vi "GOOP400_ConfigurationMemory.vi"(1 "OptionsIn":T1, 5 "error in (no error)":errorcluster, 6 "Action":enum16{"Read", "Load", "Save"}(ring)) -> (15 "OptionsOut":T1, 19 "error out":errorcluster)   [LabVIEW 2020]
uses:
  GOOP400_Options.ctl
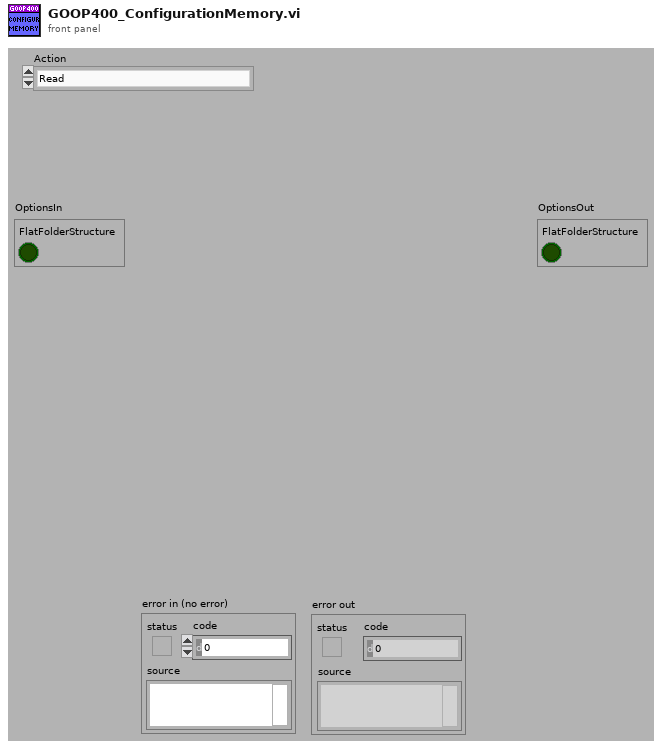
[diagram p1: front panel]
types:
  T1 = typedef "GOOP400_Options.ctl" = cluster{"FlatFolderStructure":bool}
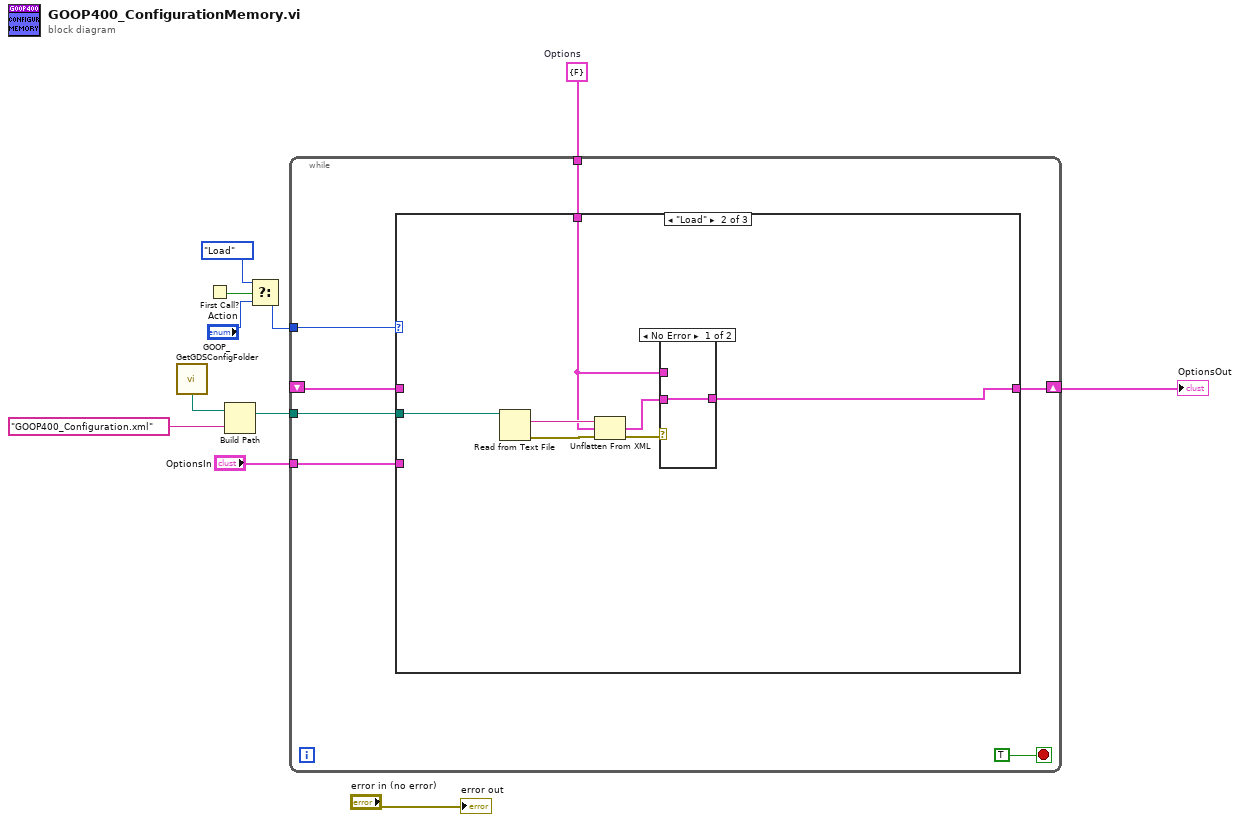
[diagram p0: block diagram]
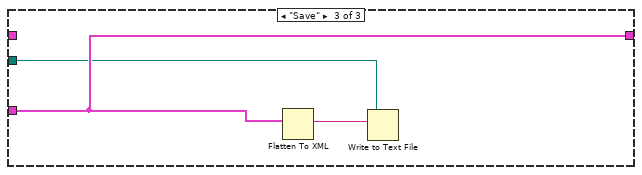
[diagram p4: hidden frame]
diagram:
  w1 = T1 {"FlatFolderStructure"=FALSE}  # Options
  n1 = call "GOOP_GetGDSConfigFolder.vi"() -> ("GDSFolderPath"=w10:path)
  n2 = First Call?() -> (First Call?: T/F=w7:bool)
  n3 = Build Path(base path=w10, name or relative path="GOOP400_Configuration.xml") -> (appended path=w9:path)
  n4 = Select(t=enum16{"Read", "Load", "Save"}."Load", s=w7, f="Action") -> (s? t:f=w5:enum16{"Read", "Load", "Save"})
  n5 = while {
    tunnel: w5 -> [w18]
    tunnel: w9 -> [w17]
    tunnel: w1 -> [w16]
    shift-right: [w14] -> w8
    shift-left: _ -> [w13]
    tunnel: "OptionsIn" -> [w12]
    stop <- TRUE stop-if-true
    n6 = case shown="\"Load\"" w18 {
      tunnel: w17 -> [_ w22 w29]
      tunnel: w16 -> [_ w21 _]
      tunnel: [w19 w20 w30] -> w14
      tunnel: w13 -> [w19 _ _]
      tunnel: w12 -> [_ _ w30]
      frame "Read", Default {
      }
      frame "Load" {
        n7 = Read from Text File(file (use dialog)=w22) -> (text=w23:string, error out=w24:errorcluster)  [unwired: 3 in, 2 out]
        n8 = Unflatten From XML(xml string=w23, type=w21, error in (no error)=w24) -> (value=w26:T1, error out=w25:errorcluster)
        n9 = case shown="No Error" w25 {
          tunnel: w26 -> [w27 _]
          tunnel: [w27 w28] -> w20
          tunnel: w21 -> [_ w28]
          frame No Error {
          }
          frame Error {
          }
        }
      }
      frame "Save" {
        n10 = Flatten To XML(6:w30) -> (2:w31:string)
        n11 = Write to Text File(file (use dialog)=w29, text=w31) -> ()  [unwired: 2 in, 3 out]
      }
    }
  }
  "OptionsOut" <- w8
  "error out" <- "error in (no error)"
